vi "Read Parameters.vi"(8 "error in (no error)":errorcluster, 11 "Selec Refn":T6) -> (0 "error out":errorcluster, 3 "Selec":T1)   [LabVIEW 2018]
uses:
  Selectors Refnums--cluster.ctl
  Digit--control.ctl
  Selectors--cluster.ctl
  Multiplier--control.ctl
  Tolerance--control.ctl
  Temp Coef--control.ctl
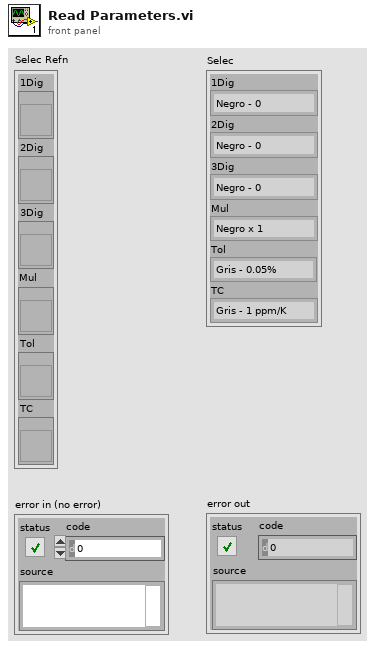
[diagram p1: front panel]
types:
  T1 = typedef "Selectors--cluster.ctl" = cluster{"1Dig":T2, "2Dig":T2, "3Dig":T2, "Mul":T3, "Tol":T4, "TC":T5}
  T2 = typedef "Digit--control.ctl" = enum16{"Negro - 0", "Marron - 1", "Rojo - 2", "Naranja - 3", "Amarillo - 4", "Verde - 5", "Azul - 6", "Violeta - 7", "Gris - 8", "Blanco - 9"}
  T3 = typedef "Multiplier--control.ctl" = enum16{"Negro x 1", "Marron x 10", "Rojo x 100", "Naranja x 1K", "Amarillo x 10K", "Verde x 100K", " Azul x 1M", "Violeta x 10M ", "Oro x 0.1", "Plata x 0.01"}
  T4 = typedef "Tolerance--control.ctl" = enum16{"Gris - 0.05%", "Violeta - 0.1%", "Azul - 0.25%", "Verde - 0.5%", "Marron - 1%", "Rojo - 2%", "Oro - 5%", "Plata - 10%", "Ninguno - 20%"}
  T5 = typedef "Temp Coef--control.ctl" = enum16{"Gris - 1 ppm/K", "Violeta - 5 ppm/K", "Azul - 10 ppm/K", "Verde - 20 ppm/K", "Amarillo - 25 ppm/K", "Naranja - 15 ppm/K", "Rojo - 50 ppm/K", "Marron - 100 ppm/K", "Negro - 250 ppm/K"}
  T6 = typedef "Selectors Refnums--cluster.ctl" = cluster{"1Dig":refnum<vi>, "2Dig":refnum<vi>, "3Dig":refnum<vi>, "Mul":refnum<vi>, "Tol":refnum<vi>, "TC":refnum<vi>}
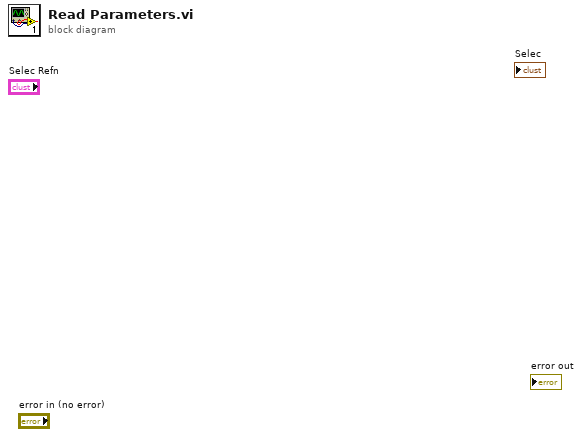
[diagram p0: block diagram]
diagram:
